vi "stack_dupn.vi"(8 "error in (no error)":errorcluster, 10 "n":i32=1, 11 "Lua in":refnum<class "Lua.lvclass">) -> (0 "error out":errorcluster, 3 "Lua out":refnum<class "Lua.lvclass">)   [LabVIEW 2020, in "Lua for LabVIEW.lvlib" / "Lua.lvclass"]
doc: "Rotates the stack elements between the valid index idx and the top of the stack. The elements are rotated n positions in the direction of the top, for a positive n, or -n positions in the direction of the bottom, for a negative n. The absolute value of n must not be greater than the size of the slice being rotated. This function cannot be called with a pseudo-index, because a pseudo-index is not an actual stack position."
uses:
  Lua.lvclass
  Lua.lvclass/Lua.ctl
  lib/lua.dll/lua.dll.lvlib
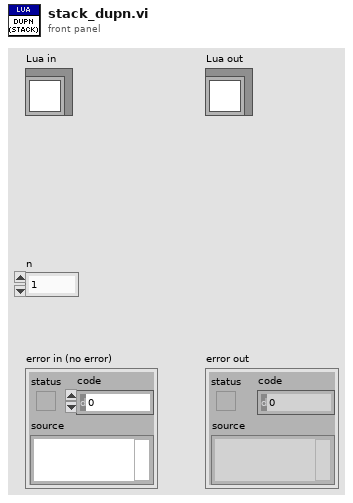
[diagram p1: front panel]
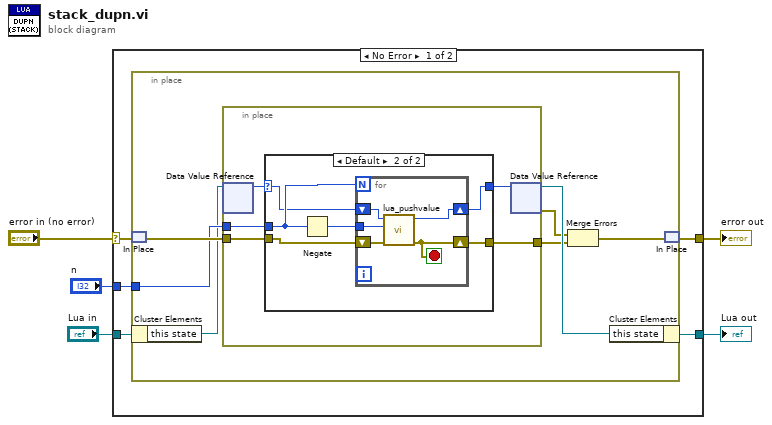
[diagram p0: block diagram]
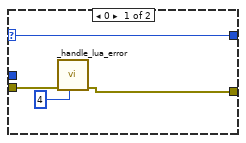
[diagram p2: hidden frame]
diagram:
  n1 = case shown="No Error" "error in (no error)" {
    selector: "error in (no error)" -> [w7 w39]
    tunnel: [w8 w39] -> w4
    tunnel: [w9 w38] -> w2
    tunnel: "Lua in" -> [w10 w38]
    tunnel: "n" -> [w6 _]
    frame No Error {
      n2 = in-place {
        in-place-border: w6 -> [w16]
        n3 = in-place-match #1(w7) -> (w17:errorcluster)
        n4 = in-place-cluster #2(w10) -> ("this state"=w14:refnum<data-value>)
        n5 = in-place {
          in-place-border: w17 -> [w22]
          in-place-border: [w21] -> w12
          in-place-border: w16 -> [w20]
          n6 = in-place-dvr #3(w14) -> (w19:u64)  [unwired: 1 out]
          n7 = case shown="Default" w19 {
            selector: w19 -> [w26 w29]
            tunnel: [w26 w28] -> w18
            tunnel: w22 -> [w23 w32]
            tunnel: [w24 w27] -> w21
            tunnel: w20 -> [_ w31]
            frame 0 {
              n8 = call "_handle_lua_error.vi"("lua status"=4 ("lua_load errcode"), "error in (no error)"=w23) -> ("error out"=w24:errorcluster)  [unwired: 9 in]
            }
            frame Default {
              n9 = Negate(x=w31) -> (-x=w30:i32)
              n10 = for {
                N: w31 -> [_]
                shift-right: [w35] -> w28
                shift-left: w29 -> [w36]
                shift-right: [w33] -> w27
                shift-left: w32 -> [w34]
                tunnel: w30 -> [w37]
                stop <- w33 stop-if-true
                n11 = call "lua_pushvalue.vi"("error in (no error)"=w34, "index"=w37, "lua_state_p"=w36) -> ("error out"=w33:errorcluster, "lua_state_p out"=w35:u64)  [unwired: 7 in]
              }
            }
          }
          n12 = in-place-dvr #3(w18) -> (w15:refnum<data-value>, w13:errorcluster)
        }
        n13 = Merge Errors(w13, w12) -> (w11:errorcluster)
        n14 = in-place-cluster #2("this state"=w15) -> (w9:refnum<class "Lua.lvclass">)
        n15 = in-place-match #1(w11) -> (w8:errorcluster)
      }
    }
    frame Error {
    }
  }
  "error out" <- w4
  "Lua out" <- w2
